vi "Scale Type.vi"(8 "error in (no error)":errorcluster, 11 "Scale in":refnum<class "Scale Config.lvclass">) -> (0 "error out":errorcluster, 2 "Scale Type":T1, 3 "Scale out":refnum<class "Scale Config.lvclass">)   [LabVIEW 2020, in "VolatusConfig.lvlib" / "Scale Config.lvclass"]
uses:
  Scale Config.lvclass
  C:/dev/lv20CE/relink/lv-volatus/VolatusConfig/VolatusConfigElement/VolatusConfigElement.lvclass
  Scale Type.ctl
  VolatusConfigElement/VolatusConfigElement.lvclass/VolatusConfigElement.ctl
  VolatusConfigElement/Element.vi
  Scale Config.lvclass/Scale Config.ctl
  VolatusConfigElement/VolatusConfigElement.lvclass
  lv-cdm/CDM-Config/Config Element/Config Element.lvclass
  VolatusConfig.lvlib
  C:/dev/lv20CE/relink/lv-volatus/VolatusConfig/Scale/Scale Config.lvclass
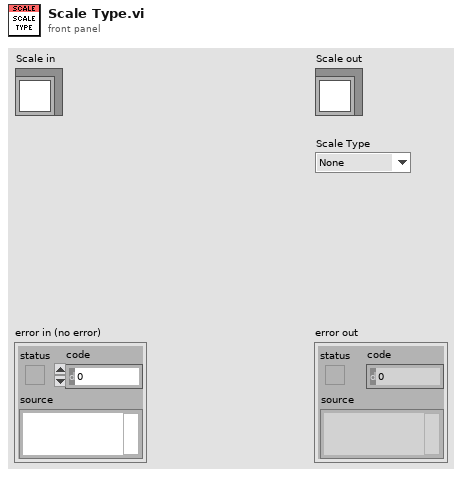
[diagram p1: front panel]
types:
  T1 = typedef "VolatusConfig.lvlib/Scale Type.ctl" = enum16{"None", "Sensor", "Polynomial", "Threshold", "Invert Bool", "Exponential"}
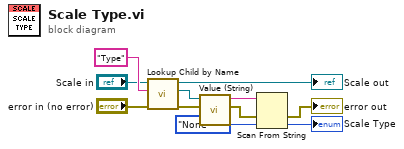
[diagram p0: block diagram]
diagram:
  n1 = call "Lookup Child by Name.vi"("error in (no error)"="error in (no error)", "Child Name"="Type", "VolatusConfigElement in"="Scale in") -> ("error out"=w10:errorcluster, "Child"=w9:refnum<class "Config Element.lvclass">, "VolatusConfigElement out"=→"Scale out":refnum<class "Scale Config.lvclass">)  [unwired: 5 in, 1 out]
  n2 = call "Value (String).vi"("error in (no error)"=w10, "Config Element in"=w9) -> ("error out"=w6:errorcluster, "String Value"=w7:string)  [unwired: 8 in]
  n3 = Scan From String(input string=w7, error in=w6, default 1=Scale_Type."None" ("Scaling Type")) -> (error out=→"error out":errorcluster, output 1=→"Scale Type":T1)  [unwired: 2 in, 2 out]
